vi "Add Sibling.vi"(8 "error in (no error)":errorcluster, 10 "Sibling":refnum<data-value>, 11 "NodeRef In":refnum<data-value>) -> (0 "error out":errorcluster, 3 "NodeRef":refnum<data-value>)   [LabVIEW 2020, in "PicoG-ParserLexer.lvlib" / "Node.lvclass"]
doc: "Adds a new sibling to the end of the current sibling list. If nodes are have the same parent (They are already siblings) then no action is taken. New sibling must not have a parent assigned already.\n\n<b>Error Codes:</b>\n<b>14</b>: New sibling already has a parent assigned. To move a node around the tree it must be removed from its parent with RemoveChild first.\n<b>1556</b>: One of the nodes is not instantiated; call Ctor for the instance first."
uses:
  Node.lvclass
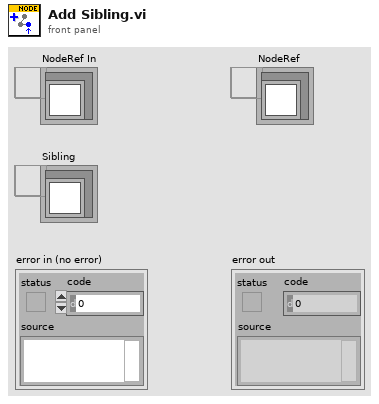
[diagram p1: front panel]
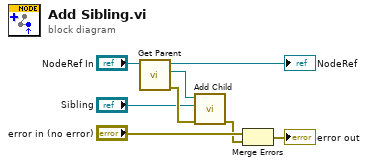
[diagram p0: block diagram]
diagram:
  n1 = call "Get Parent.vi"("NodeRef In"="NodeRef In") -> ("error out"=w8:errorcluster, "Parent"=w3:refnum<data-value>, "NodeRef"=→"NodeRef":refnum<data-value>)  [unwired: 8 in]
  n2 = call "Add Child.vi"("error in (no error)"=w8, "Child"="Sibling", "NodeRef In"=w3) -> ("error out"=w1:errorcluster)  [unwired: 7 in, 1 out]
  n3 = Merge Errors("error in (no error)", w1) -> (→"error out":errorcluster)
